vi "Test Duplicate Names for Different Assertions.vi"(8 "error in (no error)":errorcluster) -> (0 "error out":errorcluster)   [LabVIEW 2020]
uses:
  classes/Test/Test.lvclass
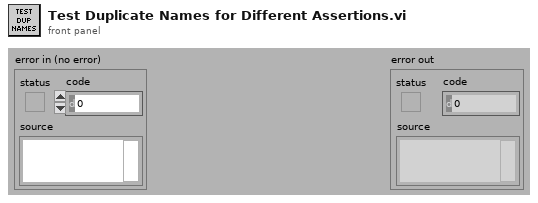
[diagram p1: front panel]
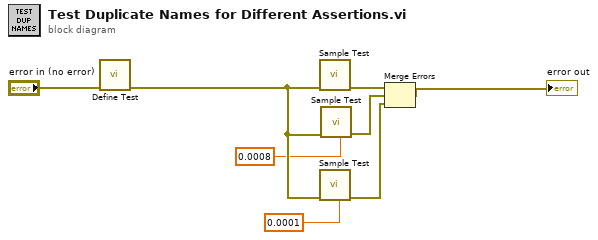
[diagram p0: block diagram]
diagram:
  n1 = call "Define Test.vi"("error in (no error)"="error in (no error)") -> ("error out"=w3:errorcluster)  [unwired: 9 in, 1 out]
  n2 = call "Sample Test.vi"("error in (no error)"=w3) -> ("error out"=w7:errorcluster)  [unwired: 10 in]
  n3 = call "Sample Test.vi"("Execution time (s)"=0.0001, "error in (no error)"=w3) -> ("error out"=w5:errorcluster)  [unwired: 9 in]
  n4 = call "Sample Test.vi"("Execution time (s)"=0.0008, "error in (no error)"=w3) -> ("error out"=w6:errorcluster)  [unwired: 9 in]
  n5 = Merge Errors(w7, w6, w5) -> (→"error out":errorcluster)
